vi "set Reference Level and Atten and Reference Offset.vi"(8 "error in (no error)":errorcluster, 10 "Reference Level, Atten, Reference Offset":T1, 11 "Keysight 9020A in":refnum<class "Keysight 9020A.lvclass">) -> (0 "error out":errorcluster, 3 "Keysight 9020A out":refnum<class "Keysight 9020A.lvclass">)   [LabVIEW 2023, in "Spectrum Analyzer.lvlib" / "Keysight 9020A.lvclass"]
uses:
  Keysight 9020A.lvclass
  TYPE DEFINITION/TYPE Reference Level and Atten Param.ctl
  Keysight 9020A.lvclass/Keysight 9020A.ctl
  Spectrum Analyzer.lvlib
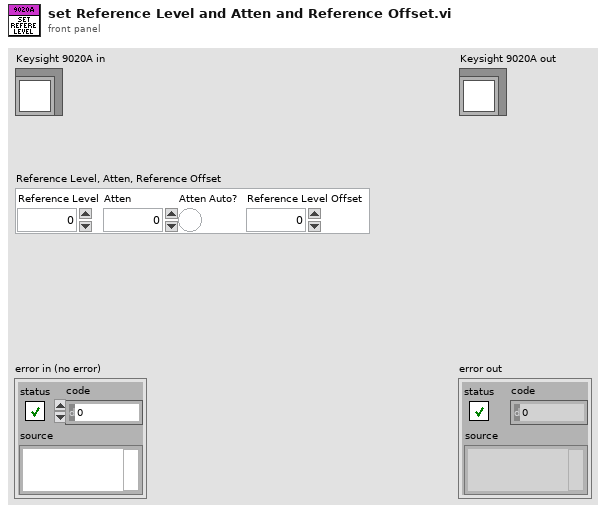
[diagram p1: front panel]
types:
  T1 = typedef "Spectrum Analyzer.lvlib/TYPE Reference Level and Atten Param.ctl" = cluster{"Reference Level":dbl, "Atten":i32, "Atten Auto?":bool, "Reference Level Offset":dbl}
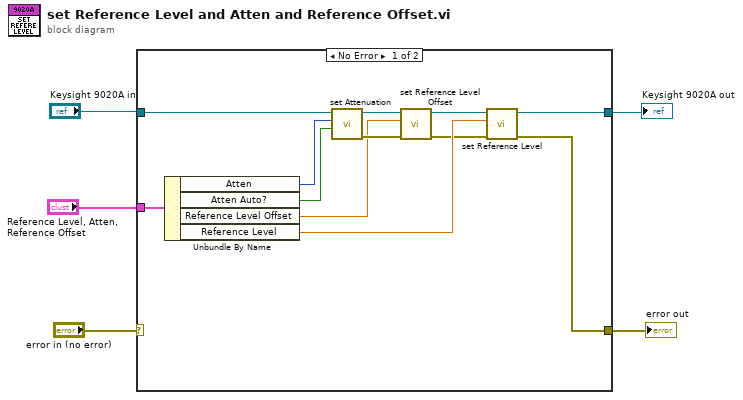
[diagram p0: block diagram]
diagram:
  n1 = case shown="No Error" "error in (no error)" {
    selector: "error in (no error)" -> [_ w18]
    tunnel: "Keysight 9020A in" -> [w14 w19]
    tunnel: [w16 w19] -> w4
    tunnel: [w15 w18] -> w1
    tunnel: "Reference Level, Atten, Reference Offset" -> [w17 _]
    frame No Error {
      n2 = Unbundle By Name(w17) -> ("Atten"=w13:i32, "Atten Auto?"=w12:bool, "Reference Level Offset"=w9:dbl, "Reference Level"=w7:dbl)
      n3 = call-dynamic "set Attenuation.vi"("Auto?"=w12, "Attenuation"=w13, "Keysight 9020A in"=w14) -> ("error out"=w10:errorcluster, "Keysight 9020A out"=w11:refnum<class "Keysight 9020A.lvclass">)  [unwired: 7 in]
      n4 = call-dynamic "set Reference Level Offset.vi"("error in (no error)"=w10, "Reference Level Offset"=w9, "Keysight 9020A in"=w11) -> ("error out"=w6:errorcluster, "Keysight 9020A out"=w8:refnum<class "Keysight 9020A.lvclass">)  [unwired: 7 in]
      n5 = call-dynamic "set Reference Level.vi"("error in (no error)"=w6, "Reference Level"=w7, "Keysight 9020A in"=w8) -> ("error out"=w15:errorcluster, "Keysight 9020A out"=w16:refnum<class "Keysight 9020A.lvclass">)  [unwired: 7 in]
    }
    frame Error {
    }
  }
  "error out" <- w1
  "Keysight 9020A out" <- w4
